vi "hamming decoder.vi"(10 "number of control bits":i32, 11 "Encoded Message":bool[](array[boolean])) -> (3 "decoded message":bool[](array[boolean]))   [LabVIEW 2025]
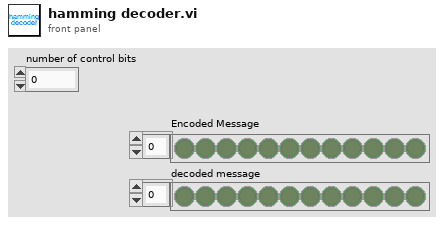
[diagram p1: front panel]
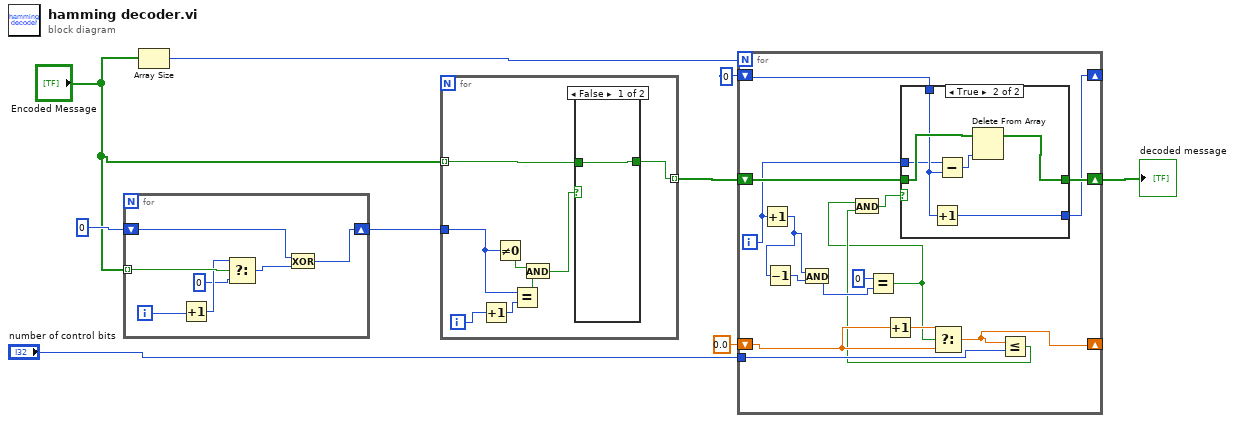
[diagram p0: block diagram]
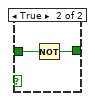
[diagram p2: hidden frame]
diagram:
  n1 = for {
    shift-right: [w10] -> w1
    shift-left: 0 -> [w11]
    tunnel: "Encoded Message" -> [w15] mode=indexing
    i -> [w16]
    n2 = Increment(x=w16) -> (x+1=w14:i32)
    n3 = Select(t=w14, s=w15, f=0) -> (s? t:f=w12:i32)
    n4 = Exclusive Or(1:w12, 2:w11) -> (0:w10:i32)
  }
  n5 = Array Size(array="Encoded Message") -> (size(s)=w7:i32)
  n6 = for {
    tunnel: [w24] -> w3 mode=indexing
    tunnel: "Encoded Message" -> [w23] mode=indexing
    tunnel: w1 -> [w22]
    i -> [w18]
    n7 = Increment(x=w18) -> (x+1=w17:i32)
    n8 = Not Equal To 0?(x=w22) -> (x != 0?=w20:bool)
    n9 = Equal?(x=w22, y=w17) -> (x = y?=w21:bool)
    n10 = And(x=w20, y=w21) -> (x .and. y?=w19:bool)
    n11 = case shown="False" w19 {
      tunnel: [w25 w26] -> w24
      tunnel: w23 -> [w25 w27]
      frame False {
      }
      frame True {
        n12 = Not(x=w27) -> (.not. x?=w26:bool)
      }
    }
  }
  n13 = for {
    N: w7 -> [_]
    shift-right: [w38] -> _
    shift-left: 0 -> [w39]
    shift-right: [w33] -> _
    shift-left: 0.0 -> [w34]
    tunnel: "number of control bits" -> [w32]
    shift-right: [w41] -> w5
    shift-left: w3 -> [w40]
    i -> [w28]
    n14 = Increment(x=w28) -> (x+1=w36:i32)
    n15 = Decrement(x=w36) -> (x-1=w37:i32)
    n16 = And(x=w36, y=w37) -> (x .and. y?=w43:i32)
    n17 = Equal?(x=0, y=w43) -> (x = y?=w29:bool)
    n18 = Increment(x=w34) -> (x+1=w35:dbl)
    n19 = Select(t=w35, s=w29, f=w34) -> (s? t:f=w33:dbl)
    n20 = Less Or Equal?(x=w33, y=w32) -> (x <= y?=w31:bool)
    n21 = And(x=w29, y=w31) -> (x .and. y?=w30:bool)
    n22 = case shown="True" w30 {
      tunnel: [w44 w49] -> w41
      tunnel: w40 -> [w44 w50]
      tunnel: w39 -> [w45 w48]
      tunnel: [w45 w51] -> w38
      tunnel: w28 -> [_ w46]
      frame False {
      }
      frame True {
        n23 = Increment(x=w48) -> (x+1=w51:i32)
        n24 = Subtract(x=w46, y=w48) -> (x-y=w47:i32)
        n25 = Delete From Array(array=w50, index=w47) -> (array with subset deleted=w49:bool[])  [unwired: 1 in, 1 out]
      }
    }
  }
  "decoded message" <- w5
